vi "BNO055correction.vi"() -> ()   [LabVIEW 2019]
uses:
  <vilib>/Utility/error.llb/Error Cluster From Error Code.vi
  <vilib>/myRIO/Common/Instrument Driver Framework/myRIO v1.0/I2C/vis/myRIO v1.0 Write I2C.vi
  <vilib>/myRIO/Common/Instrument Driver Framework/myRIO v1.0/I2C/vis/myRIO v1.0 Read I2C.vi
  <vilib>/Platform/TimedLoop/XDataNode/XDataNode.xnode
  <vilib>/Platform/TimedLoop/XDataNode/nitl_modes.ctl
  <vilib>/Platform/TimedLoop/XDataNode/XDNodeRunTimeDep.lvlib
  <vilib>/Platform/TimedLoop/XDataNode/wakeup.ctl
  <vilib>/Platform/TimedLoop/XDataNode/timing_clust.ctl
  GlobalVariable.vi
  <vilib>/myRIO/Instrument Drivers/Onboard IO/I2C/I2C.lvlib
panel:
  out "Array":dbl[](array[numeric])
  out "x+y":dbl
  out "x-y":dbl
  out "Bytes Read":u8[](array[numeric])=[159, 5, 245, 255, 244, 255]
  out "x/y":cluster{"Yaw":dbl, "Roll":dbl, "Pitch":dbl}={"Yaw"=89.9375, "Roll"=-0.6875, "Pitch"=-0.75}
  out "error out 2":errorcluster
  in  "reset":bool
  in  "disabled":bool
  out "result":dbl[](array[numeric])=[0.1875, 0.1875, 0.1875]
  in  "value":dbl=1.0
  in  "目標":dbl[](array[numeric])=[0.0, 0.0, 0.0] format="%#_13g"
  in  "error in (no error) 2":errorcluster
  in  "Numeric":dbl
  out "out":dbl[](array[numeric])=[0.1875, 0.1875, 0.1875]
  in  "error in (no error)":errorcluster
  out "error":dbl=0.0625
  in  "stop":bool
  out "error out":errorcluster
  in  "degree":dbl=90.0
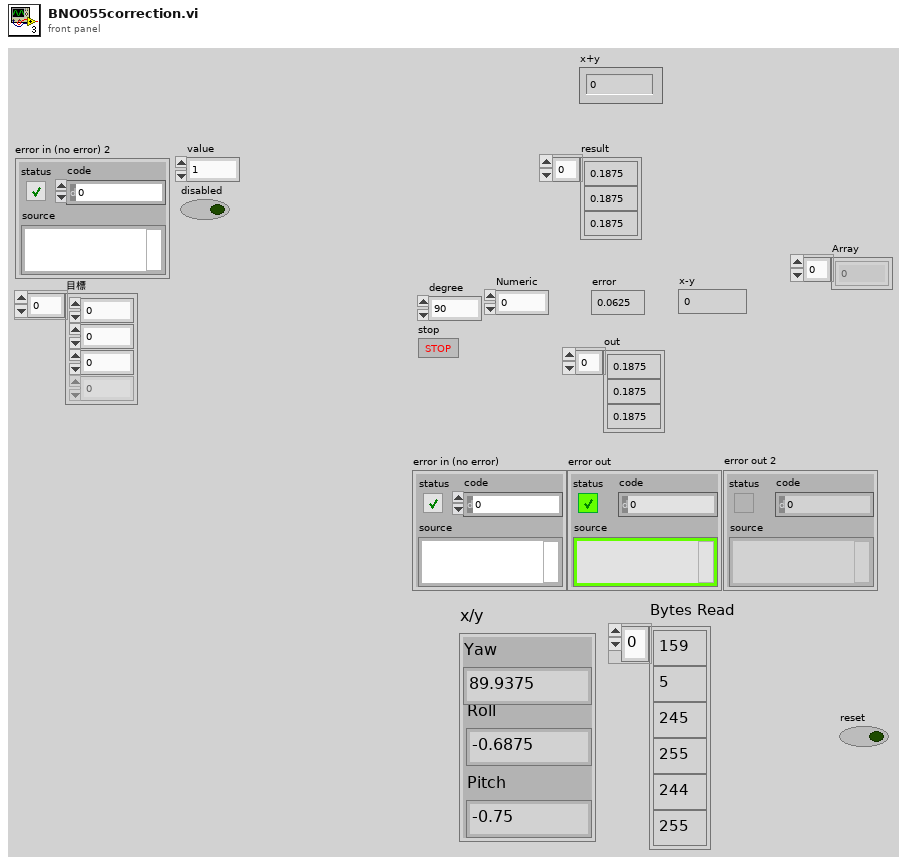
[diagram p1: front panel]
types:
  T1 = typedef "XDNodeRunTimeDep.lvlib/timing_clust.ctl" = cluster{"Expected End [f-1]":u64, "Actual End [f-1]":u64, "Finished Late? [f-1]":bool, "Expected End [i-1]":u64, "Actual End [i-1]":u64, "Finished Late? [i-1]":bool, "Expected Start [i]":u64, "Actual Start [i]":u64, "Expected Start [f]":u64, "Actual Start [f]":u64, "Source Name":string, "Structure Name":string, "Period":i64, "Deadline":i64, "Offset":i64, "Start":i64, "Priority":i32, "Timeout":i32, "Mode":T2, "Wakeup Reason":T3, "Error":errorcluster, "Source Type":string, "Secondary Source Type":string, "Global End Time":u64, "Global Start Time":u64, "Frame Duration":u64, "Iteration Duration":u64, "Assigned CPU":i32, "I/O Scan Engine Mode":u32}
  T2 = typedef "XDNodeRunTimeDep.lvlib/nitl_modes.ctl" = enum32{"No Change", "Process missed periods, maintain original phase", "Discard missed periods, maintain original phase", "Process missed periods, ignore original phase", "Discard missed periods, ignore original phase"}
  T3 = typedef "XDNodeRunTimeDep.lvlib/wakeup.ctl" = enum32{"Normal", "Aborted", "Asynchronous wakeup", "Timing source error", "Timed loop error", "Timeout"}
  T4 = typedef "I2C.lvlib/I2C Reference.ctl" = cluster{"myRIO Reference":T5, "I2C Channels Enum":T9, "I2C Configuration":T10}
  T5 = typedef "myRIO Generic Hardware Reference.ctl" = cluster{"myRIO Model":T6, "myRIO Hardware Reference":T7}
  T6 = typedef "Hardware Version Enum.ctl" = enum16{"Unknown", "myRIO-1900", "myRIO-1950", "roboRIO", "NI ELVIS RIO CM", "ELVIS III"}
  T7 = typedef "myRIO v1.0 Reference.ctl" = cluster{"Generic FPGA Reference":T8, "Allow multiple opens":bool}
  T8 = typedef "Generic FPGA Reference.ctl" = refnum<k20>
  T9 = typedef "I2C Channels Enum.ctl" = enum16{"Not Connected", "A/I2C", "B/I2C", "I2C/I2C"}
  T10 = typedef "I2C.lvlib/I2C Configuration.ctl" = cluster{"I2C Transfer Rate":T11}
  T11 = typedef "I2C.lvlib/I2C Transfer Rate.ctl" = enum16{"Standard mode (100 kbps)", "Fast mode (400 kbps)"}
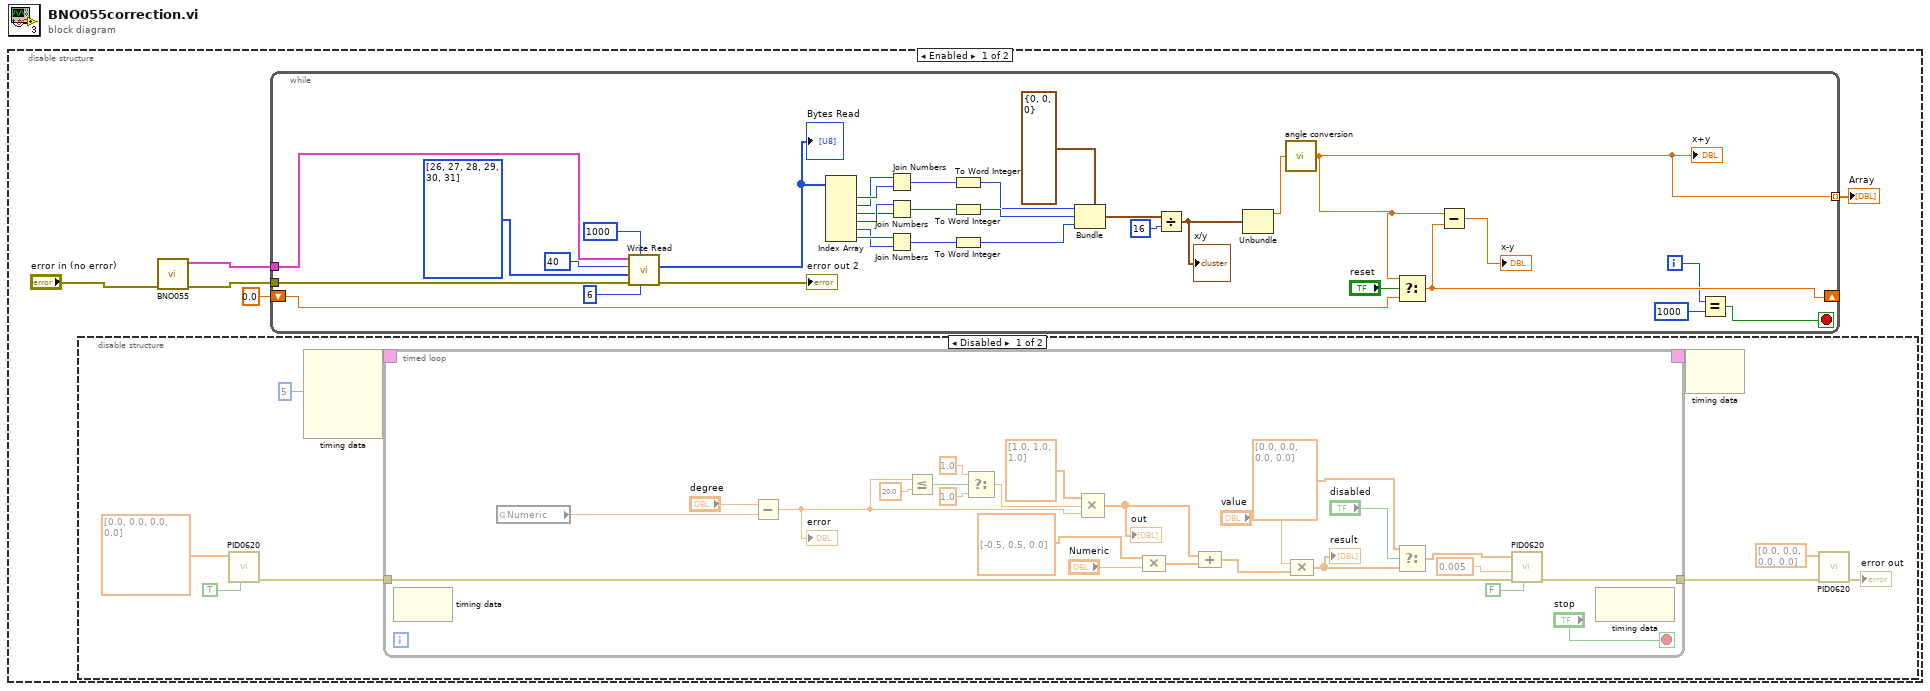
[diagram p0: block diagram]
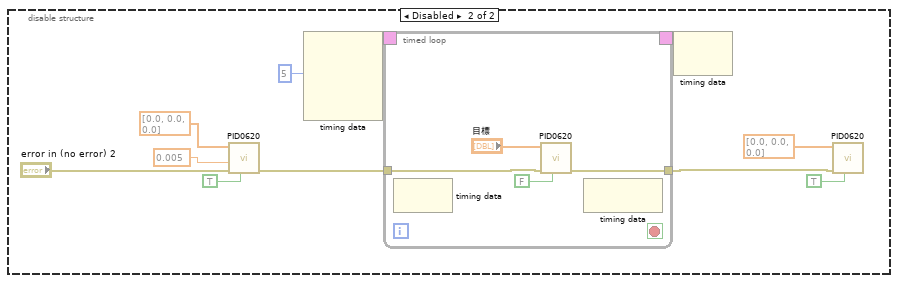
[diagram p3: hidden frame]
diagram:
  n1 = disable-structure shown="Enabled" {
    frame Enabled {
      n2 = disable-structure shown="Disabled" {
        frame Disabled {
          n3 = call "PID0620.vi"("Reset Counter"=TRUE, "目標"=dbl[] [0.0, 0.0, 0.0, 0.0]) -> ("error out"=w7:errorcluster, "error in (no error)"=w6:errorcluster)  [unwired: 8 in]
          n4 = node-c288(i64 5 ("Period")) -> (w15:T1)  [unwired: 3 in]
          n5 = timed-loop {
            tunnel: [w24] -> w11
            timing: w15 -> [_]
            timing-out: [_] -> w14
            tunnel: w7 -> [w25]
            stop <- "stop" stop-if-true
            n6 = node-c288() -> ()  [unwired: 1 in, 1 out]
            n7 = global read "GlobalVariable.vi" "Numeric"() -> (w37:dbl)
            n8 = Subtract(x="degree", y=w37) -> (x-y=w31:dbl)
            "error" <- w31
            n9 = Less Or Equal?(x=w31, y=20.0) -> (x <= y?=w29:bool)
            n10 = Select(t=1.0 ("value"), s=w29, f=1.0) -> (s? t:f=w26:dbl)
            n11 = Compound Arithmetic op=MULTIPLY(dbl[] [1.0, 1.0, 1.0] ("value"), w26, w31) -> (w34:dbl[])
            "out" <- w34
            n12 = Compound Arithmetic op=MULTIPLY(dbl[] [-0.5, 0.5, 0.0] ("value"), "Numeric") -> (w33:dbl[])
            n13 = Compound Arithmetic op=ADD(w34, w33) -> (w23:dbl[])
            n14 = Compound Arithmetic op=MULTIPLY("value", w23) -> (w19:dbl[])
            "result" <- w19
            n15 = Select(t=dbl[] [0.0, 0.0, 0.0, 0.0] ("目標"), s="disabled", f=w19) -> (s? t:f=w16:dbl[])
            n16 = call "PID0620.vi"("Reset Counter"=FALSE, "error in (no error)"=w25, "dt (s)"=0.005, "目標"=w16) -> ("error out"=w24:errorcluster)  [unwired: 7 in]
            n17 = node-c288() -> ()  [unwired: 1 in, 1 out]
          }
          n18 = node-c288(w14) -> ()  [unwired: 1 out]
          n19 = call "PID0620.vi"("error in (no error)"=w11, "目標"=dbl[] [0.0, 0.0, 0.0, 0.0]) -> ("error out"=→"error out":errorcluster)  [unwired: 9 in]
        }
        frame Enabled {
        }
      }
      n20 = call "BNO055.vi"("error in (no error)"="error in (no error)") -> ("error out"=w3:errorcluster, "I2C Ref Out"=w2:T4)  [unwired: 9 in]
      n21 = while {
        tunnel: w3 -> [w78]
        tunnel: w2 -> [w77]
        shift-right: [w53] -> _
        shift-left: 0.0 -> [w54]
        tunnel: [w46] -> w1 mode=indexing
        i -> [w49]
        stop <- w47 stop-if-true
        n22 = call <vilib>:"Write Read.vi"("Byte Count"=u32 6, "Timeout ms (1000)"=1000, "error in (no error)"=w78, "Bytes to Write"=i32[] [26, 27, 28, 29, 30, 31], "Slave Address (7-bit)"=40, "I2C Ref In"=w77) -> ("error out"=→"error out 2":errorcluster, "Bytes Read"=w72:u8[])  [unwired: 2 in, 1 out]
        "Bytes Read" <- w72
        n23 = Index Array(array=w72) -> (element #1=w60:u8, element #2=w55:u8, element #3=w66:u8, element #4=w67:u8, element #5=w64:u8, element #6=w65:u8)  [unwired: 6 in]
        n24 = Join Numbers(hi=w55, lo=w60) -> ((hi.lo)=w63:u16)
        n25 = Join Numbers(hi=w67, lo=w66) -> ((hi.lo)=w62:u16)
        n26 = Join Numbers(hi=w65, lo=w64) -> ((hi.lo)=w61:u16)
        n27 = To Word Integer(number=w63) -> (16bit integer=w56:i16)
        n28 = To Word Integer(number=w62) -> (16bit integer=w71:i16)
        n29 = To Word Integer(number=w61) -> (16bit integer=w70:i16)
        n30 = Bundle(cluster=cluster{"Yaw":i16, "Roll":i16, "Pitch":i16} {"Yaw"=0, "Roll"=0, "Pitch"=0}, "Yaw"=w56, "Roll"=w71, "Pitch"=w70) -> (w69:cluster{"Yaw":i16, "Roll":i16, "Pitch":i16})
        n31 = Divide(x=w69, y=u32 16 ("Byte Count")) -> (x/y=w57:cluster{"Yaw":dbl, "Roll":dbl, "Pitch":dbl})
        "x/y" <- w57
        n32 = Unbundle(w57) -> ("Yaw"=w50:dbl)  [unwired: 2 out]
        n33 = call "angle conversion.vi"("Numeric Control"=w50) -> ("x+y"=w46:dbl)
        "x+y" <- w46
        n34 = Select(t=w46, s="reset", f=w54) -> (s? t:f=w53:dbl)
        n35 = Subtract(x=w46, y=w53) -> (x-y=→"x-y":dbl)
        n36 = Equal?(x=w49, y=1000) -> (x = y?=w47:bool)
      }
      "Array" <- w1
    }
    frame Disabled {
      n37 = call "PID0620.vi"("Reset Counter"=TRUE, "error in (no error)"="error in (no error) 2", "dt (s)"=0.005, "目標"=dbl[] [0.0, 0.0, 0.0]) -> ("error out"=w86:errorcluster)  [unwired: 7 in]
      n38 = node-c288(i64 5 ("Period")) -> (w89:T1)  [unwired: 3 in]
      n39 = timed-loop {
        timing: w89 -> [_]
        timing-out: [_] -> w88
        tunnel: w86 -> [w93]
        tunnel: [w92] -> w85
        stop <- _ stop-if-true
        n40 = node-c288() -> ()  [unwired: 1 in, 1 out]
        n41 = call "PID0620.vi"("Reset Counter"=FALSE, "error in (no error)"=w93, "目標"="目標") -> ("error out"=w92:errorcluster)  [unwired: 8 in]
        n42 = node-c288() -> ()  [unwired: 1 in, 1 out]
      }
      n43 = node-c288(w88) -> ()  [unwired: 1 out]
      n44 = call "PID0620.vi"("Reset Counter"=TRUE, "error in (no error)"=w85, "目標"=dbl[] [0.0, 0.0, 0.0]) -> ()  [unwired: 8 in, 1 out]
    }
  }
